vi "Status Policy.vi"(9 "failures in":u32, 10 "state":string, 11 "call error":errorcluster) -> (0 "error out":errorcluster, 2 "update status":bool, 3 "failures out":u32)   [LabVIEW 2021, in "CAN RW CANsub.lvclass"]
doc: "Decides what Update CAN Status does with the result of a status call. A failed call gives no error and counts up; 12 failures in a row give error 5303. A good call resets the count; the state \"stopped\" gives error 5304. Loop-safe when no error is made: no allocation, bounded time."
uses:
  CAN RW CANsub.lvclass
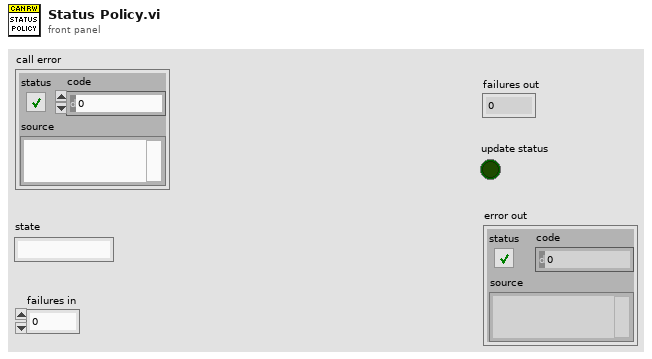
[diagram p1: front panel]
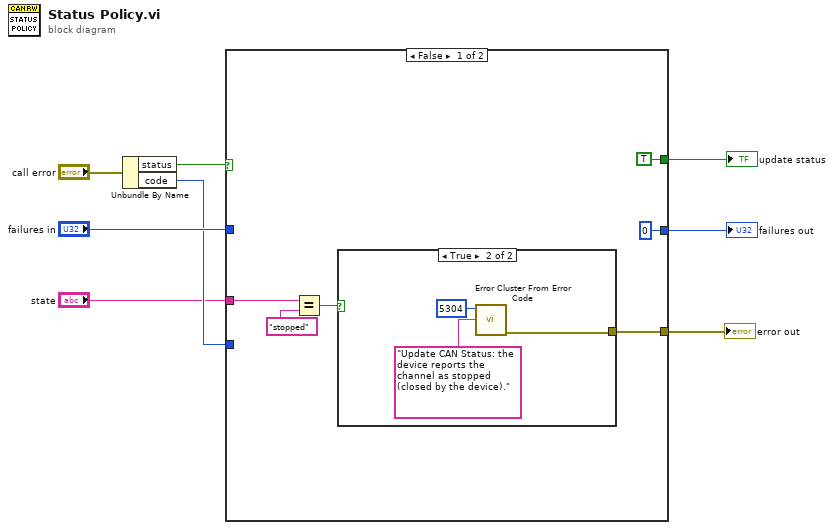
[diagram p0: block diagram]
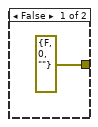
[diagram p2: hidden frame]
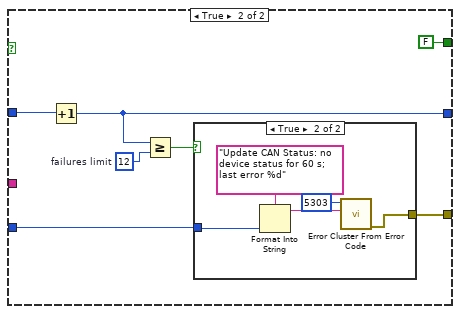
[diagram p3: hidden frame]
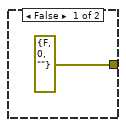
[diagram p4: hidden frame]
diagram:
  n1 = Unbundle By Name("call error") -> ("status"=w7:bool, "code"=w2:i32)
  n2 = case shown="False" w7 {
    tunnel: "failures in" -> [_ w25]
    tunnel: [u32 0 w23] -> w5
    tunnel: [TRUE FALSE] -> w4
    tunnel: [w9 w20] -> w3
    tunnel: w2 -> [_ w19]
    tunnel: "state" -> [w12 _]
    frame False {
      n3 = Equal?(x=w12, y="stopped") -> (x = y?=w10:bool)
      n4 = case shown="True" w10 {
        tunnel: [errorcluster {"status"=FALSE, "code"=0, "source"=""} ("error constant") w18] -> w9
        frame False {
        }
        frame True {
          n5 = call <vilib>:"Error Cluster From Error Code.vi"("error message (\"\")"="Update CAN Status: the device reports the channel as stopped (closed by the device).", "error code (0)"=5304) -> ("error out"=w18:errorcluster)  [unwired: 7 in]
        }
      }
    }
    frame True {
      w22 = u32 12  # failures limit
      n6 = Increment(x=w25) -> (x+1=w23:u32)
      n7 = Greater Or Equal?(x=w23, y=w22) -> (x >= y?=w21:bool)
      n8 = case shown="True" w21 {
        tunnel: [errorcluster {"status"=FALSE, "code"=0, "source"=""} ("error constant") w27] -> w20
        tunnel: w19 -> [_ w30]
        frame False {
        }
        frame True {
          n9 = Format Into String(format string="Update CAN Status: no device status for 60 s; last error %d", w30) -> (resulting string=w28:string)  [unwired: 2 in, 1 out]
          n10 = call <vilib>:"Error Cluster From Error Code.vi"("error message (\"\")"=w28, "error code (0)"=5303) -> ("error out"=w27:errorcluster)  [unwired: 7 in]
        }
      }
    }
  }
  "update status" <- w4
  "failures out" <- w5
  "error out" <- w3
